vi "Test - Draw Filled Triangle.vi"() -> ()   [LabVIEW 2020, in "Raster.lvlib"]
uses:
  Raster.lvlib
  Utility/Utility.lvlib
  Rectangle Dimensions.ctl
  5ea285c7-be76-47ab-bb95-511c6a9aac96.vi
  d84cddbd-8e40-43c7-a758-6e8d8fd6f2c6.vi
  3D/Vector 3D.ctl
  3D/3D.lvlib
  UV.ctl
  3D/Vertex.ctl
  3D/Triangle.ctl
  Texture.ctl
  3D/Material.ctl
panel:
  in  "Triangle":T1={"Vertex 1"={"Position"={"x"=75.0, "y"=25.0, "z"=0.0}, "UV"={"u"=0.0, "v"=0.0}, "Colour"=12517256}, "Vertex 2"={"Position"={"x"=500.0, "y"=450.0, "z"=0.0}, "UV"={"u"=0.0, "v"=0.0}, "Colour"=12517256}, "Vertex 3"={"Position"={"x"=50.0, "y"=200.0, "z"=0.0}, "UV"={"u"=0.0, "v"=0.0}, "Colour"=12517256}, "Alpha"=0.0, "Alpha Blending Enabled"=FALSE, "Colour"=10092492, "Material"={"Diffuse Colour"=0, "Texture"={"Pixels"=refnum, "Size"={"Width"=0, "Height"=0}}}} {"Vertex 3"."UV"."v" min=0 max=1 step=0.1; "Vertex 3"."UV"."u" min=0 max=1 step=0.1; "Vertex 2"."UV"."v" min=0 max=1 step=0.1; "Vertex 2"."UV"."u" min=0 max=1 step=0.1; "Vertex 1"."UV"."v" min=0 max=1 step=0.1; "Vertex 1"."UV"."u" min=0 max=1 step=0.1}
  out "Time [s]":dbl format="%.3p"
  out "new picture":picture
  # "(0,0)"
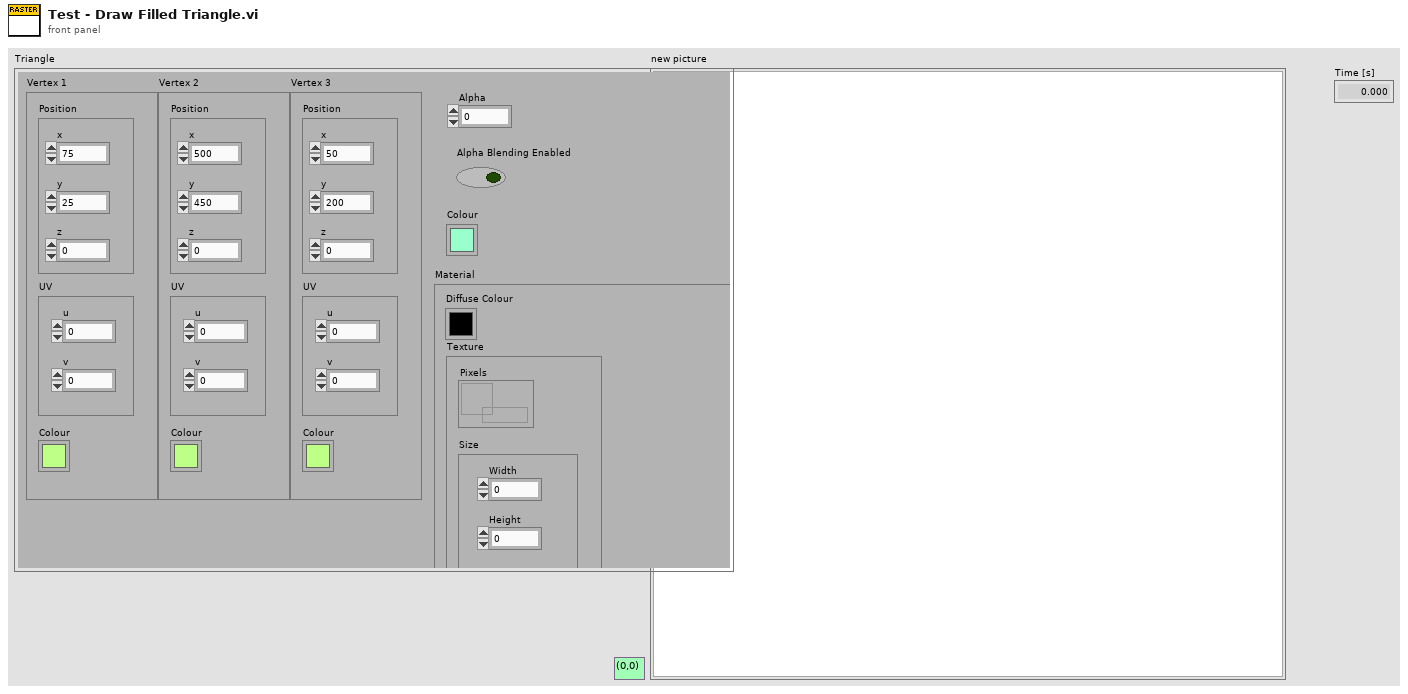
[diagram p1: front panel]
types:
  T1 = typedef "3D.lvlib/Triangle.ctl" = cluster{"Vertex 1":T2, "Vertex 2":T2, "Vertex 3":T2, "Alpha":dbl, "Alpha Blending Enabled":bool, "Colour":u32, "Material":T5}
  T2 = typedef "3D.lvlib/Vertex.ctl" = cluster{"Position":T3, "UV":T4, "Colour":u32}
  T3 = typedef "3D.lvlib/Vector 3D.ctl" = cluster{"x":sgl, "y":sgl, "z":sgl}
  T4 = typedef "Raster.lvlib/UV.ctl" = cluster{"u":sgl, "v":sgl}
  T5 = typedef "3D.lvlib/Material.ctl" = cluster{"Diffuse Colour":u32, "Texture":T6}
  T6 = typedef "Raster.lvlib/Texture.ctl" = cluster{"Pixels":refnum<data-value>, "Size":T7}
  T7 = typedef "Raster.lvlib/Rectangle Dimensions.ctl" = cluster{"Width":u32, "Height":u32}
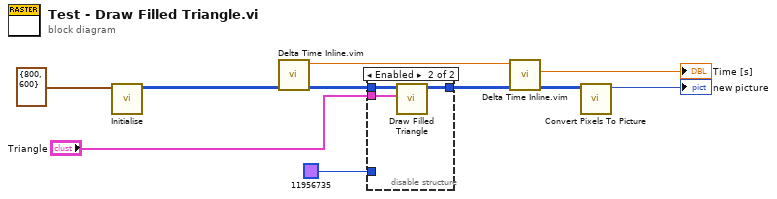
[diagram p0: block diagram]
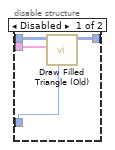
[diagram p2: hidden frame]
diagram:
  n1 = call "Initialise.vi"("Screen Dimensions"=T7 {"Width"=800, "Height"=600}) -> ("Pixel Data out"=w7:u32[][])  [unwired: 10 in]
  n2 = call "Delta Time Inline.vim"("value in"=w7) -> ("value out"=w6:u32[][], "Relative Seconds out [s]"=w2:dbl)  [unwired: 8 in, 1 out]
  n3 = disable-structure shown="Enabled" {
    disable-tunnel: u32 11956735 ("Line Colour") -> [w14 _]
    disable-tunnel: w6 -> [w13 w17]
    disable-tunnel: [w12 w16] -> w5
    disable-tunnel: "Triangle" -> [w11 w15]
    frame Disabled {
      n4 = call "Draw Filled Triangle (Old).vi"(6:w14, "Triangle"=w11, "Pixel Data in"=w13) -> ("Pixel Data out"=w12:u32[][])  [unwired: 8 in]
    }
    frame Enabled {
      n5 = call "Draw Filled Triangle.vi"("Triangle"=w15, "Pixel Data in"=w17) -> ("Pixel Data out"=w16:u32[][])  [unwired: 9 in]
    }
  }
  n6 = call "Delta Time Inline.vim"("value in"=w5, "Relative Seconds in [s]"=w2) -> ("value out"=w4:u32[][], "Delta Time [s]"=→"Time [s]":dbl)  [unwired: 7 in, 1 out]
  n7 = call "Convert Pixels To Picture.vi"("Pixel Data in"=w4) -> ("2D Picture"=→"new picture":picture)  [unwired: 9 in, 1 out]
